vi "ZM-PC-getDataAsJson.vi"(8 "error in (no error)":errorcluster, 11 "ZM-PC-EP-error_package in":refnum<class "ZM-PC-EP-error_package.lvclass">) -> (0 "error out":errorcluster, 2 "json":string, 3 "ZM-PC-EP-error_package out":refnum<class "ZM-PC-EP-error_package.lvclass">)   [LabVIEW 2020, in "ZM-PC-packages.lvlib" / "ZM-PC-EP-error_package.lvclass"]
doc: "Error-package override of getDataAsJson (dynamic dispatch, own body, no Call Parent): the header strings from the parent's getHeader and the data cluster from Read data, bundled as {timestamp, type, destination, data} and flattened to JSON with LabVIEW extensions off. The data keys are sender, code, source."
uses:
  ZM-PC-EP-error_package.lvclass
  ZM-PC-EP-error_package.lvclass/ZM-PC-EP-error_package.ctl
  ZM-PC-package/ZM-PC-package.lvclass
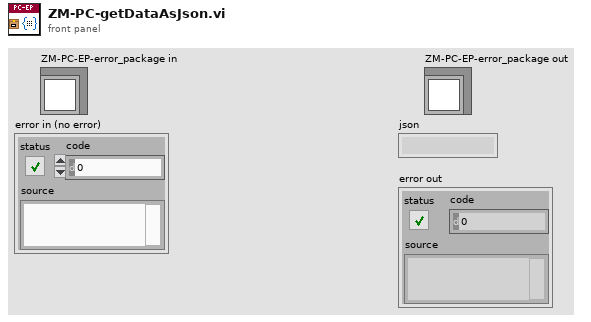
[diagram p1: front panel]
types:
  T1 = cluster{"timestamp":string, "type":string, "destination":string, "data":cluster{"sender":string, "code":i32, "source":string}}
  T2 = typedef "ZM-PC-packages.lvlib/ZM-PC-package.lvclass/ZM-PC-HEADER.ctl" = cluster{"timestamp":string, "type":string, "destination":string}
  T3 = typedef "ZM-PC-packages.lvlib/ZM-PC-EP-error_package.lvclass/ZM-PC-EP-DATA.ctl" = cluster{"sender":string, "code":i32, "source":string}
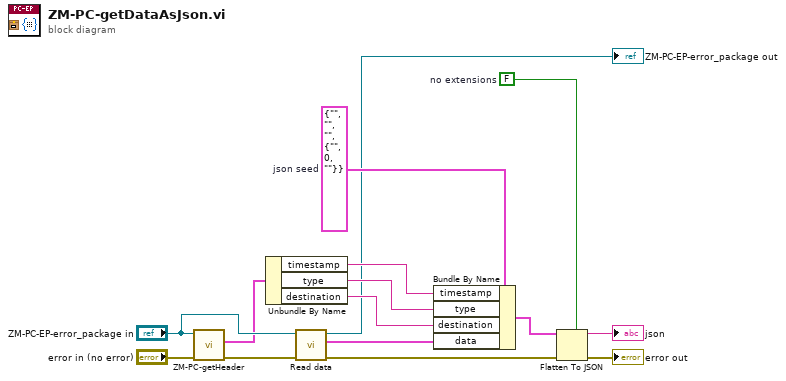
[diagram p0: block diagram]
diagram:
  w4 = FALSE  # no extensions
  w7 = T1 {"timestamp"="", "type"="", "destination"="", "data"={"sender"="", "code"=0, "source"=""}}  # json seed
  n1 = call "ZM-PC-getHeader.vi"("error in (no error)"="error in (no error)", "ZM-PC-package in"="ZM-PC-EP-error_package in") -> ("error out"=w14:errorcluster, "header"=w12:T2)  [unwired: 7 in, 1 out]
  n2 = Unbundle By Name(w12) -> ("timestamp"=w11:string, "type"=w10:string, "destination"=w9:string)
  n3 = call "Read data.vi"("error in (no error)"=w14, "ZM-PC-EP-error_package in"="ZM-PC-EP-error_package in") -> ("error out"=w5:errorcluster, "ZM-PC-EP-DATA"=w8:T3, "ZM-PC-EP-error_package out"=→"ZM-PC-EP-error_package out":refnum<class "ZM-PC-EP-error_package.lvclass">)  [unwired: 7 in]
  n4 = Bundle By Name(cluster=w7, "timestamp"=w11, "type"=w10, "destination"=w9, "data"=w8) -> (w6:T1)
  n5 = Flatten To JSON(enable LabVIEW extensions? (T)=w4, anything=w6, error in (no error)=w5) -> (JSON string=→"json":string, 11:→"error out":errorcluster)
